vi "_nicrio_cRIO-9217_UpdateControls.vi"(0 "D":refnum<vi>, 1 "C":refnum<vi>, 2 "B":refnum<vi>, 3 "A":refnum<vi>, 4 "9217 Config":T1 {"RTD_Type" items=["TCR3851"=1, "TCR3750"=2, "TCR3916"=3, "TCR3920"=4, "TCR3911"=5, "TCR3928"=6, "Custom"=0]; "Degree Range" items=["Raw Ohms", "Degrees Kelvin", "Degrees Celsius", "Degrees Fahrenheit", "Degrees Rankine"]; "Conversion Time" items=["200 ms", "2.5 ms"]}, 5 "TypeControl":refnum<vi>, 6 "Values":i32[](array[numeric])=[0], 7 "TypeTypeDef":refnum<vi>, 8 "RTD Type":u8, 9 "Units":u8, 10 "UnitsControl":refnum<vi>, 11 "UnitsTypeDef":refnum<vi>) -> ()   [LabVIEW 2020, in "Modules.lvlib" / "9217.lvclass"]
uses:
  9217.lvclass
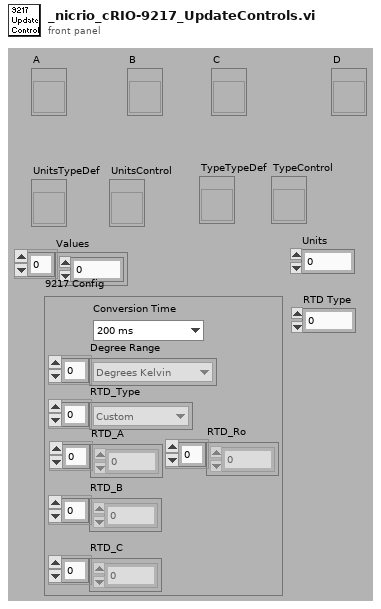
[diagram p1: front panel]
types:
  T1 = cluster{"Conversion Time":u16, "Degree Range":u8[], "RTD_Type":u8[], "RTD_A":dbl[], "RTD_B":dbl[], "RTD_C":dbl[], "RTD_Ro":dbl[]}
  T2 = typedef "LVStringsAndValuesArrayTypeDef_U8.ctl" = cluster{"String":string, "Value":u8}[]
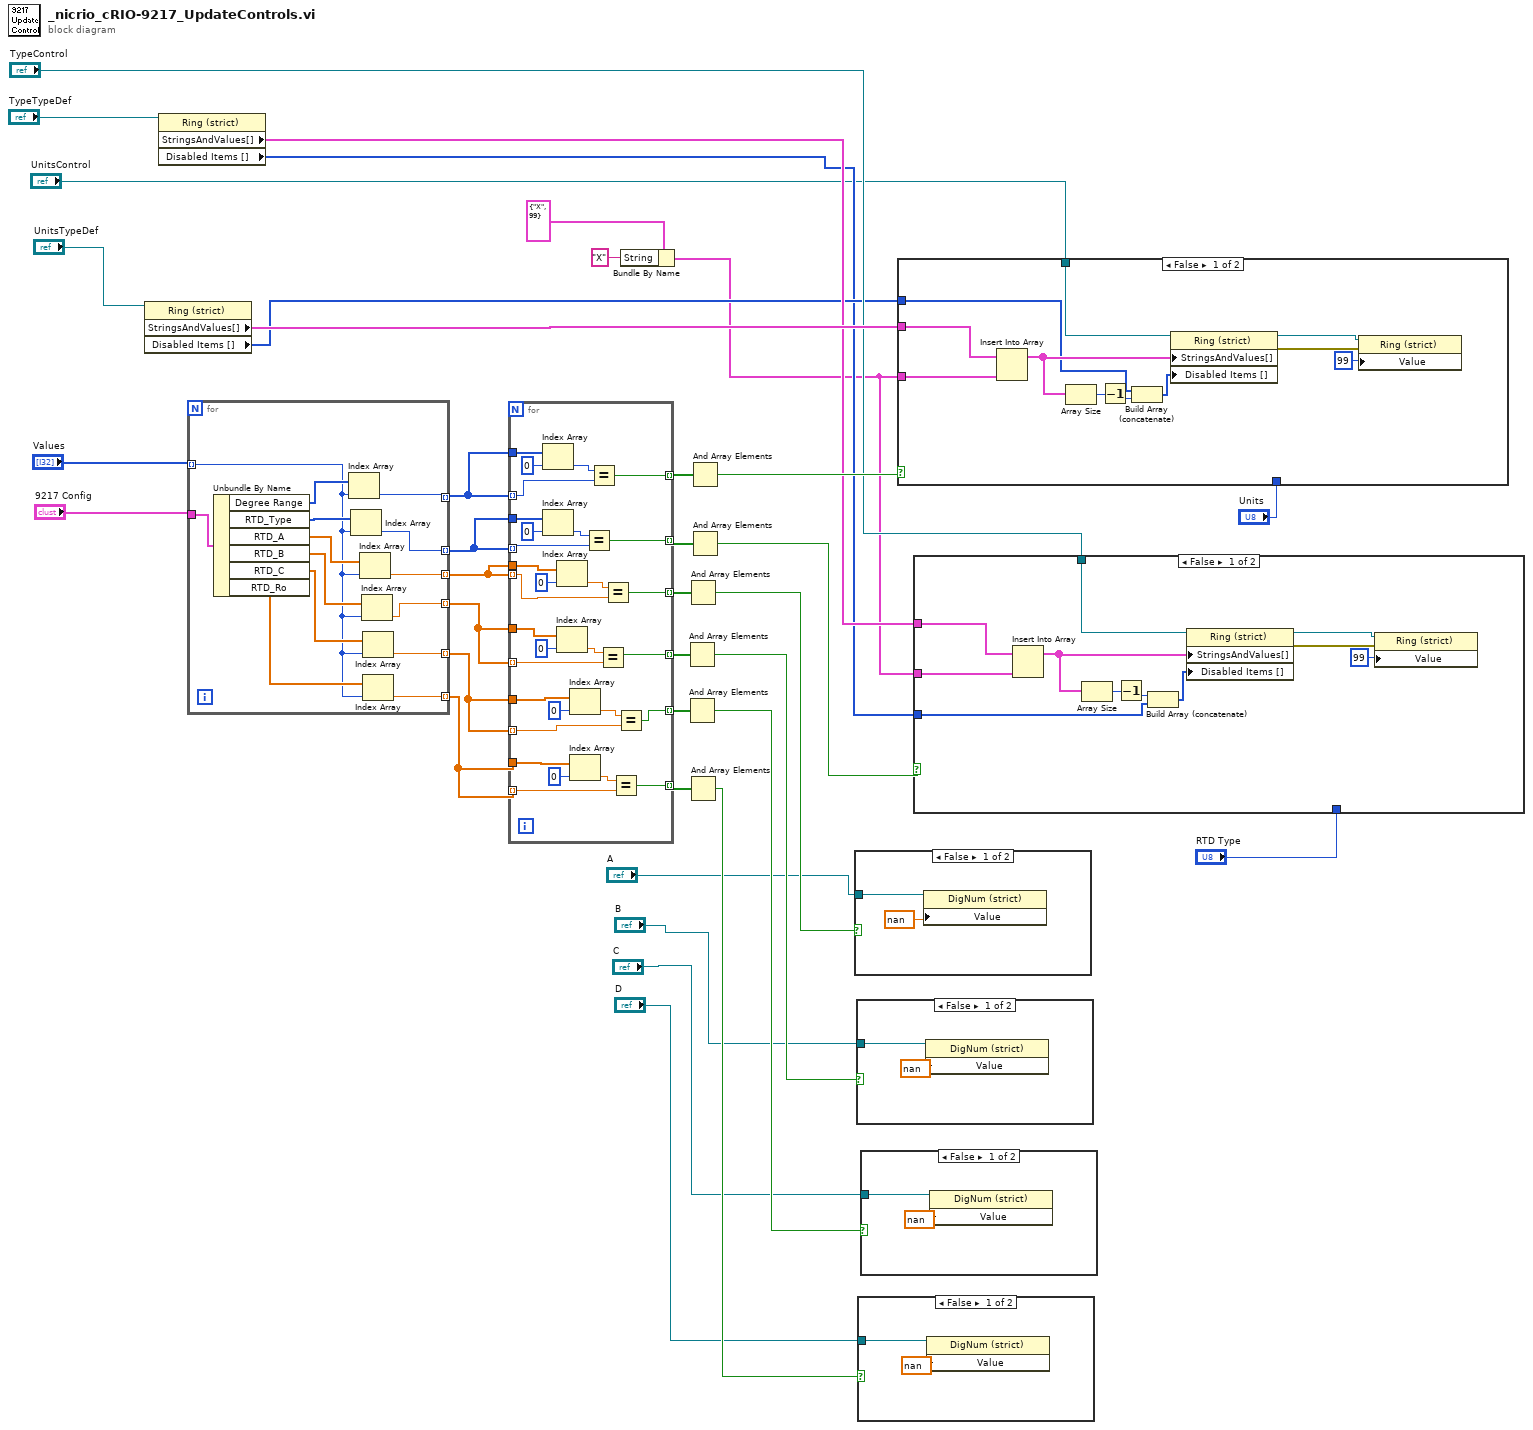
[diagram p0: block diagram]
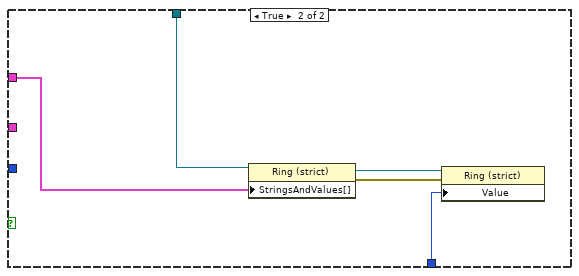
[diagram p6: hidden frame]
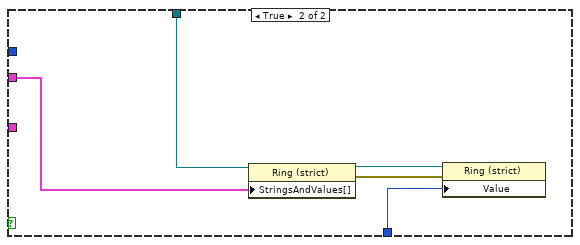
[diagram p7: hidden frame]
diagram:
  n1 = property on="Property Node" class="Ring (strict)"(reference="UnitsTypeDef") -> ("StringsAndValues[]"=w30:T2, "Disabled Items []"=w9:i32[])  [unwired: 1 in, 2 out]
  n2 = property on="Property Node" class="Ring (strict)"(reference="TypeTypeDef") -> ("StringsAndValues[]"=w27:T2, "Disabled Items []"=w8:i32[])  [unwired: 1 in, 2 out]
  n3 = for {
    tunnel: "Values" -> [w42] mode=indexing
    tunnel: "9217 Config" -> [w51]
    tunnel: [w48] -> w35 mode=indexing
    tunnel: [w47] -> w34 mode=indexing
    tunnel: [w41] -> w22 mode=indexing
    tunnel: [w40] -> w23 mode=indexing
    tunnel: [w39] -> w24 mode=indexing
    tunnel: [w38] -> w25 mode=indexing
    n4 = Unbundle By Name(w51) -> ("Degree Range"=w50:u8[], "RTD_Type"=w49:u8[], "RTD_A"=w46:dbl[], "RTD_B"=w45:dbl[], "RTD_C"=w44:dbl[], "RTD_Ro"=w43:dbl[])
    n5 = Index Array(array=w50, index=w42) -> (element=w48:u8)
    n6 = Index Array(array=w49, index=w42) -> (element=w47:u8)
    n7 = Index Array(array=w46, index=w42) -> (element=w41:dbl)
    n8 = Index Array(array=w45, index=w42) -> (element=w40:dbl)
    n9 = Index Array(array=w44, index=w42) -> (element=w39:dbl)
    n10 = Index Array(array=w43, index=w42) -> (element=w38:dbl)
  }
  n11 = for {
    tunnel: w35 -> [w76] mode=indexing
    tunnel: w34 -> [w74] mode=indexing
    tunnel: w35 -> [w81]
    tunnel: w34 -> [w80]
    tunnel: [w73] -> w32 mode=indexing
    tunnel: [w72] -> w33 mode=indexing
    tunnel: w22 -> [w63] mode=indexing
    tunnel: w23 -> [w62] mode=indexing
    tunnel: w24 -> [w61] mode=indexing
    tunnel: w25 -> [w60] mode=indexing
    tunnel: w25 -> [w59]
    tunnel: w24 -> [w58]
    tunnel: w23 -> [w57]
    tunnel: w22 -> [w56]
    tunnel: [w55] -> w21 mode=indexing
    tunnel: [w54] -> w20 mode=indexing
    tunnel: [w53] -> w19 mode=indexing
    tunnel: [w52] -> w18 mode=indexing
    n12 = Index Array(array=w81, index=0) -> (element=w77:u8)
    n13 = Index Array(array=w80, index=0) -> (element=w75:u8)
    n14 = Index Array(array=w56, index=0) -> (element=w70:dbl)
    n15 = Index Array(array=w57, index=0) -> (element=w71:dbl)
    n16 = Index Array(array=w58, index=0) -> (element=w65:dbl)
    n17 = Index Array(array=w59, index=0) -> (element=w64:dbl)
    n18 = Equal?(x=w75, y=w74) -> (x = y?=w73:bool)
    n19 = Equal?(x=w77, y=w76) -> (x = y?=w72:bool)
    n20 = Equal?(x=w71, y=w62) -> (x = y?=w53:bool)
    n21 = Equal?(x=w70, y=w63) -> (x = y?=w52:bool)
    n22 = Equal?(x=w64, y=w60) -> (x = y?=w55:bool)
    n23 = Equal?(x=w65, y=w61) -> (x = y?=w54:bool)
  }
  n24 = Bundle By Name(cluster=cluster{"String":string, "Value":u8} {"String"="X", "Value"=99} ("new element/subarray"), "String"="X" ("String ID")) -> (w6:cluster{"String":string, "Value":u8})
  n25 = And Array Elements(Boolean array=w19) -> (logical AND=w16:bool)
  n26 = And Array Elements(Boolean array=w20) -> (logical AND=w15:bool)
  n27 = And Array Elements(Boolean array=w18) -> (logical AND=w17:bool)
  n28 = And Array Elements(Boolean array=w21) -> (logical AND=w14:bool)
  n29 = And Array Elements(Boolean array=w33) -> (logical AND=w31:bool)
  n30 = And Array Elements(Boolean array=w32) -> (logical AND=w29:bool)
  n31 = case shown="False" w17 {
    tunnel: "A" -> [w82 _]
    frame False {
      n32 = property on="Property Node" class="DigNum (strict)"(reference=w82, "Value"=nan) -> ()  [unwired: 1 in, 2 out]
    }
    frame True {
    }
  }
  n33 = case shown="False" w16 {
    tunnel: "B" -> [w84 _]
    frame False {
      n34 = property on="Property Node" class="DigNum (strict)"(reference=w84, "Value"=nan) -> ()  [unwired: 1 in, 2 out]
    }
    frame True {
    }
  }
  n35 = case shown="False" w14 {
    tunnel: "D" -> [w86 _]
    frame False {
      n36 = property on="Property Node" class="DigNum (strict)"(reference=w86, "Value"=nan) -> ()  [unwired: 1 in, 2 out]
    }
    frame True {
    }
  }
  n37 = case shown="False" w15 {
    tunnel: "C" -> [w88 _]
    frame False {
      n38 = property on="Property Node" class="DigNum (strict)"(reference=w88, "Value"=nan) -> ()  [unwired: 1 in, 2 out]
    }
    frame True {
    }
  }
  n39 = case shown="False" w31 {
    tunnel: w30 -> [w100 w105]
    tunnel: "UnitsControl" -> [w99 w104]
    tunnel: w9 -> [w91 _]
    tunnel: w6 -> [w90 _]
    tunnel: "Units" -> [_ w101]
    frame False {
      n40 = Insert Into Array(array=w100, new element=w90) -> (w95:T2)  [unwired: 1 in]
      n41 = Array Size(array=w95) -> (size(s)=w94:i32)
      n42 = Decrement(x=w94) -> (x-1=w93:i32)
      n43 = Build Array (concatenate)(w91, w93) -> (w92:i32[])
      n44 = property on="Property Node" class="Ring (strict)"(reference=w99, "StringsAndValues[]"=w95, "Disabled Items []"=w92) -> (reference out=w98:refnum<vi>, error out=w97:errorcluster)  [unwired: 1 in]
      n45 = property on="Property Node" class="Ring (strict)"(reference=w98, error in=w97, "Value"=u8 99) -> ()  [unwired: 2 out]
    }
    frame True {
      n46 = property on="Property Node" class="Ring (strict)"(reference=w104, "StringsAndValues[]"=w105) -> (reference out=w103:refnum<vi>, error out=w102:errorcluster)  [unwired: 1 in]
      n47 = property on="Property Node" class="Ring (strict)"(reference=w103, error in=w102, "Value"=w101) -> ()  [unwired: 2 out]
    }
  }
  n48 = case shown="False" w29 {
    tunnel: w27 -> [w116 w121]
    tunnel: "TypeControl" -> [w115 w120]
    tunnel: w8 -> [w107 _]
    tunnel: w6 -> [w106 _]
    tunnel: "RTD Type" -> [_ w117]
    frame False {
      n49 = Insert Into Array(array=w116, new element=w106) -> (w111:T2)  [unwired: 1 in]
      n50 = Array Size(array=w111) -> (size(s)=w110:i32)
      n51 = Decrement(x=w110) -> (x-1=w109:i32)
      n52 = Build Array (concatenate)(w109, w107) -> (w108:i32[])
      n53 = property on="Property Node" class="Ring (strict)"(reference=w115, "StringsAndValues[]"=w111, "Disabled Items []"=w108) -> (reference out=w114:refnum<vi>, error out=w113:errorcluster)  [unwired: 1 in]
      n54 = property on="Property Node" class="Ring (strict)"(reference=w114, error in=w113, "Value"=u8 99) -> ()  [unwired: 2 out]
    }
    frame True {
      n55 = property on="Property Node" class="Ring (strict)"(reference=w120, "StringsAndValues[]"=w121) -> (reference out=w119:refnum<vi>, error out=w118:errorcluster)  [unwired: 1 in]
      n56 = property on="Property Node" class="Ring (strict)"(reference=w119, error in=w118, "Value"=w117) -> ()  [unwired: 2 out]
    }
  }
